vi "tp_filtre.vi"(8 "error in (no error)":errorcluster, 10 "ID Query (True)":bool=TRUE, 11 "VISA resource name":refnum<visa-resource-name>) -> (0 "error out":errorcluster, 3 "VISA resource name out":refnum<visa-resource-name>)   [LabVIEW 2012]
doc: "Establishes communication with the instrument and optionally performs an instrument identification query and/or an instrument reset. It also places the instrument in a default state needed for other instrument driver operations. Therefore, call this VI before calling other instrument driver VIs for this instrument. Generally, you need to call the <B>Initialize VI</B> only once at the beginning of an application."
uses:
  <instrlib>/Agilent 34401/Agilent 34401.lvlib
panel:
  out "x = y?":bool
  # "(c) 2005-2008 National Instruments.  ALL RIGHTS RESERVED."
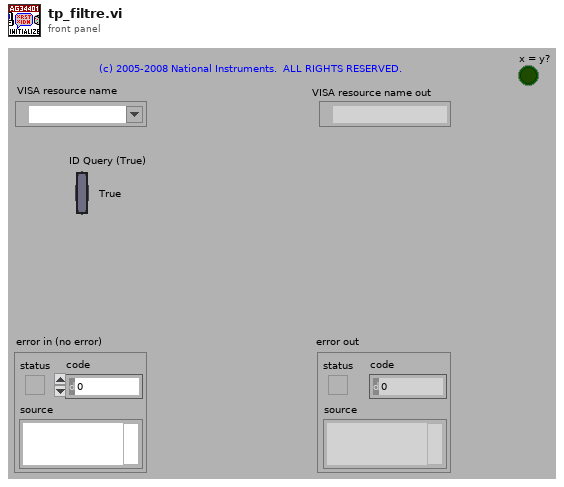
[diagram p1: front panel]
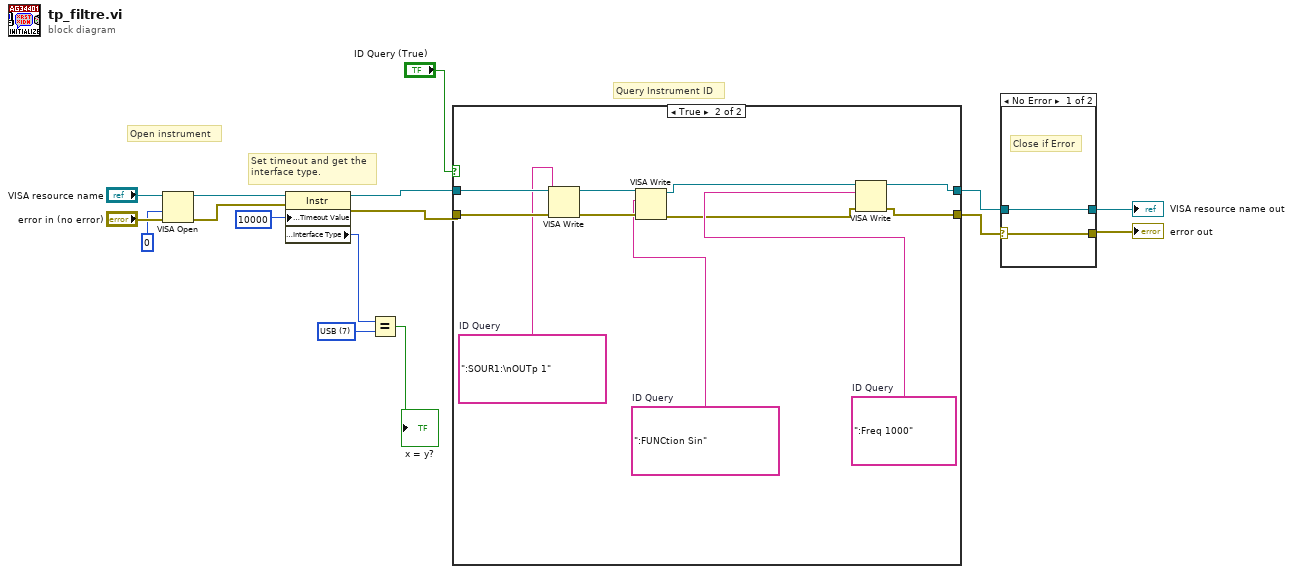
[diagram p0: block diagram]
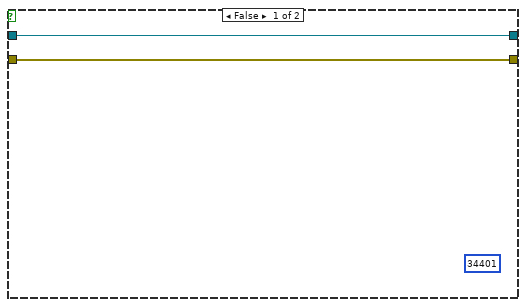
[diagram p2: hidden frame]
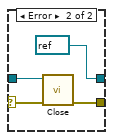
[diagram p3: hidden frame]
diagram:
  w12 = u16 7 items=["GPIB"=1, "VXI"=2, "GPIB-VXI"=3, "Serial"=4, "PXI"=5, "TCPIP"=6, "USB"=7] ("Interface Information:Interface Type")
  # "Set timeout and get the\ninterface type."
  # "Close if Error"
  # "Query Instrument ID"
  # "Open instrument"
  n1 = VISA Open(access mode=u32 0, error in (no error)="error in (no error)", VISA resource name="VISA resource name") -> (VISA resource name=w7:refnum<visa-resource-name>, error out=w6:errorcluster)  [unwired: 2 in]
  n2 = property on="Property Node" class="Instr"(reference=w7, error in=w6, "General Settings:Timeout Value"=u32 10000) -> (reference out=w5:refnum<visa-resource-name>, error out=w4:errorcluster, "Interface Information:Interface Type"=w14:u16)
  n3 = Equal?(x=w14, y=w12) -> (x = y?=→"x = y?":bool)
  n4 = case shown="True" "ID Query (True)" {
    tunnel: [w17 w19] -> w2
    tunnel: [w18 w25] -> w3
    tunnel: w5 -> [w18 w28]
    tunnel: w4 -> [w17 w29]
    frame False {
      (unwired) 34401
    }
    frame True {
      w22 = ":FUNCtion Sin"  # ID Query
      w26 = ":Freq 1000"  # ID Query
      w27 = ":SOUR1:\nOUTp 1"  # ID Query
      n5 = VISA Write(VISA resource name=w28, write buffer=w27, error in (no error)=w29) -> (VISA resource name out=w24:refnum<visa-resource-name>, error out=w23:errorcluster)  [unwired: 1 out]
      n6 = VISA Write(VISA resource name=w24, write buffer=w22, error in (no error)=w23) -> (VISA resource name out=w21:refnum<visa-resource-name>, error out=w20:errorcluster)  [unwired: 1 out]
      n7 = VISA Write(VISA resource name=w21, write buffer=w26, error in (no error)=w20) -> (VISA resource name out=w25:refnum<visa-resource-name>, error out=w19:errorcluster)  [unwired: 1 out]
    }
  }
  n8 = case shown="No Error" w2 {
    selector: w2 -> [w30 w33]
    tunnel: w3 -> [w31 w34]
    tunnel: [w31 refnum<visa-resource-name> refnum ("VISA resource name out")] -> w10
    tunnel: [w30 w35] -> w8
    frame No Error {
    }
    frame Error {
      n9 = call <instrlib>:"Close.vi"("error in (no error)"=w33, "VISA resource name"=w34) -> ("error out"=w35:errorcluster)  [unwired: 9 in]
    }
  }
  "VISA resource name out" <- w10
  "error out" <- w8
